vi "ConvertTextBasedCodeToLabVIEW_CreateInterfaceList.vi"(11 "Classes":T1[](array[typedef])) -> (3 "InterfaceItems":T13[](array[typedef]))   [LabVIEW 2020]
uses:
  ConvertTextBasedCodeToLabVIEW_MissingType.ctl
  ConvertTextBasedCodeToLabVIEW_MissingTypeIconType.ctl
  String/GDSString_ClassDescriptionType.ctl
  String/GDSString_AccessScopeModifierType.ctl
  String/GDSString_ModifierType.ctl
  String/GDSString_MethodDescriptionType.ctl
  CommonVIs/CommonVIs_AttributeType.ctl
  CommonVIs/CommonVIs_AttributeDataType.ctl
  CommonVIs/CommonVIs_PropertyType.ctl
  String/GDSString_ClassParentType.ctl
  String/GDSString_ClassType.ctl
  String/GDSString_ClassOwnerType.ctl
  CommonVIs/CommonVIs_EnumType.ctl
  CommonVIs/CommonVIs_StructType.ctl
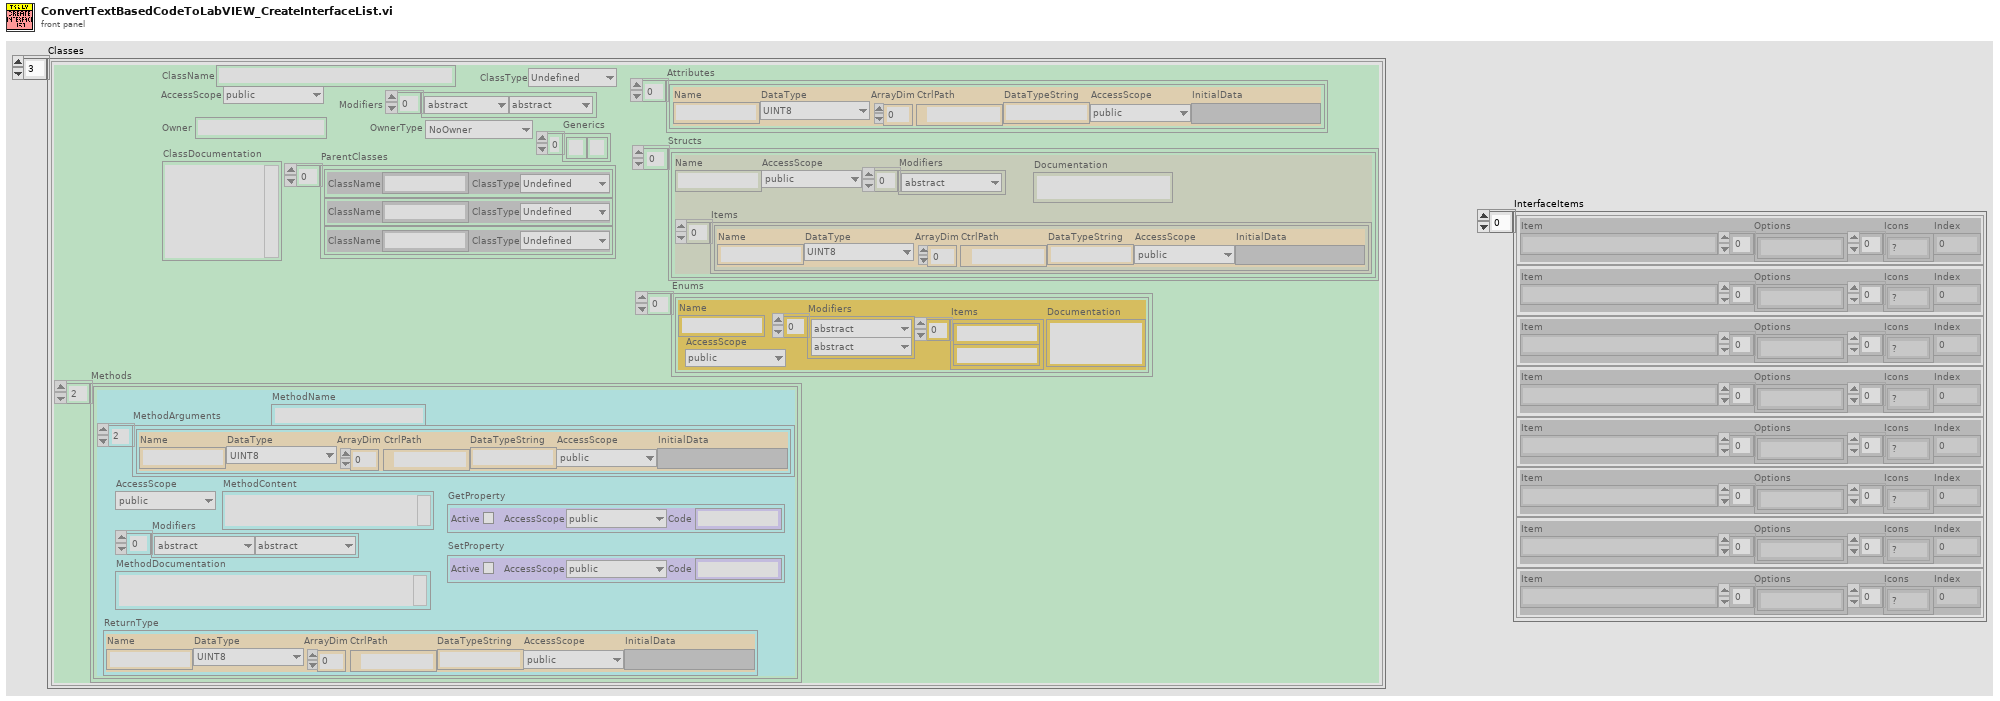
[diagram p1: front panel]
types:
  T1 = typedef "GDSString_ClassDescriptionType.ctl" = cluster{"ClassName":string, "AccessScope":T2, "Modifiers":T3[], "ClassDocumentation":string, "Methods":T4[], "ParentClasses":T8[], "ClassType":T9, "Owner":string, "OwnerType":T10, "Generics":string[], "Attributes":T5[], "Enums":T11[], "Structs":T12[]}
  T2 = typedef "GDSString_AccessScopeModifierType.ctl" = enum16{"public", "private", "protected", "internal"}
  T3 = typedef "GDSString_ModifierType.ctl" = enum16{"abstract", "static", "final", "synchronized", "strictfp", "async", "const", "event", "extern", "new", "native ", "override", "partial", "readonly", "sealed", "unsafe", "virtual", "volatile"}
  T4 = typedef "GDSString_MethodDescriptionType.ctl" = cluster{"ReturnType":T5, "MethodName":string, "AccessScope":T2, "Modifiers":T3[], "MethodDocumentation":string, "MethodContent":string, "MethodArguments":T5[], "GetProperty":T7, "SetProperty":T7}
  T5 = typedef "CommonVIs_AttributeType.ctl" = cluster{"Name":string, "DataType":T6, "ArrayDim":i32, "CtrlPath":path, "DataTypeString":string, "AccessScope":T2, "InitialData":variant}
  T6 = typedef "CommonVIs_AttributeDataType.ctl" = enum16{"UINT8", "INT8", "UINT16", "INT16", "UINT32", "INT32", "UINT64", "INT64", "SGL", "DBL", "EXT", "CSG", "CDB", "CXT", "TimeStamp", "STRING", "PATH", "BOOL", "ENUM", "RefNum", "VIRefNum", "LabVIEW Class", "Cluster", "Variant", "TypeDef", "Waveform", "LabVIEW Object", "Other", "void", "Set", "Map"}
  T7 = typedef "CommonVIs_PropertyType.ctl" = cluster{"Active":bool, "AccessScope":T2, "Code":string}
  T8 = typedef "GDSString_ClassParentType.ctl" = cluster{"ClassName":string, "ClassType":T9}
  T9 = typedef "GDSString_ClassType.ctl" = enum16{"Undefined", "Class", "Interface"}
  T10 = typedef "GDSString_ClassOwnerType.ctl" = enum16{"NoOwner", "Class", "Package/NameSpace"}
  T11 = typedef "CommonVIs_EnumType.ctl" = cluster{"Name":string, "AccessScope":T2, "Modifiers":T3[], "Items":string[], "Documentation":string}
  T12 = typedef "CommonVIs_StructType.ctl" = cluster{"Name":string, "AccessScope":T2, "Modifiers":T3[], "Items":T5[], "Documentation":string}
  T13 = typedef "ConvertTextBasedCodeToLabVIEW_MissingType.ctl" = cluster{"Item":string, "Options":string[], "Icons":T14[], "Index":i32}
  T14 = typedef "ConvertTextBasedCodeToLabVIEW_MissingTypeIconType.ctl" = enum16{"?", "Add", "Delete", "Implement", "Inherit"}
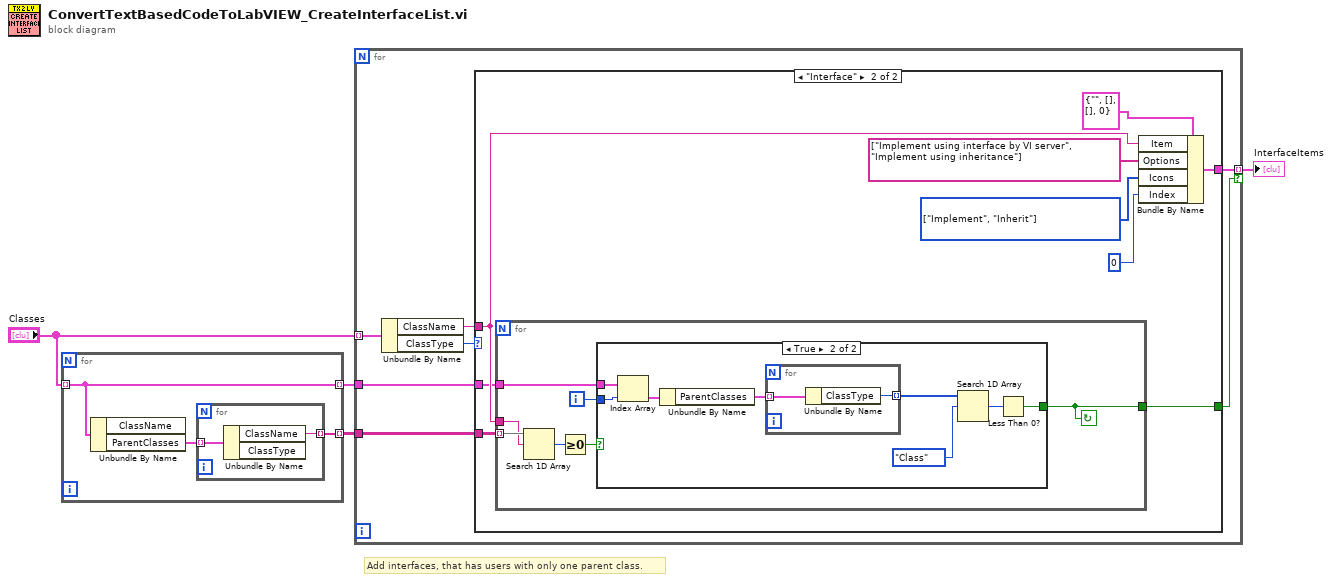
[diagram p0: block diagram]
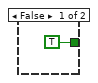
[diagram p3: hidden frame]
diagram:
  # "Add interfaces, that has users with only one parent class."
  n1 = for {
    tunnel: "Classes" -> [w5] mode=indexing
    tunnel: [w6] -> w3 mode=indexing
    tunnel: [w5] -> w2 mode=indexing
    n2 = Unbundle By Name(w5) -> ("ParentClasses"=w7:T8[])  [unwired: 1 out]
    n3 = for {
      tunnel: w7 -> [w9] mode=indexing
      tunnel: [w8] -> w6 mode=indexing
      n4 = Unbundle By Name(w9) -> ("ClassName"=w8:string)  [unwired: 1 out]
    }
  }
  n5 = for {
    tunnel: "Classes" -> [w16] mode=indexing
    tunnel: w3 -> [w13]
    tunnel: w2 -> [w12]
    tunnel: [w11] -> w1 mode=indexing if=w10
    n6 = Unbundle By Name(w16) -> ("ClassName"=w14:string, "ClassType"=w15:T9)
    n7 = case shown="\"Interface\"" w15 {
      tunnel: w14 -> [_ w20]
      tunnel: w13 -> [_ w21]
      tunnel: w12 -> [_ w19]
      tunnel: [_ w18] -> w11
      tunnel: [_ w17] -> w10
      frame Default {
      }
      frame "Interface" {
        w23 = T14[] [enum."Implement", enum."Inherit"] items=["?", "Add", "Delete", "Implement", "Inherit"] ("Icons")
        n8 = for {
          tunnel: w21 -> [w32] mode=indexing
          tunnel: w20 -> [w31]
          tunnel: w19 -> [w29]
          tunnel: [w26] -> w17
          i -> [w27]
          stop <- w26 continue-if-true
          n9 = Search 1D Array(1D array=w32, element=w31) -> (index of element=w28:i32)  [unwired: 1 in]
          n10 = Greater Or Equal To 0?(x=w28) -> (x >= 0?=w30:bool)
          n11 = case shown="True" w30 {
            tunnel: w29 -> [_ w41]
            tunnel: w27 -> [_ w40]
            tunnel: [TRUE w34] -> w26
            frame False {
            }
            frame True {
              n12 = Index Array(array=w41, index=w40) -> (element=w39:T1)
              n13 = Unbundle By Name(w39) -> ("ParentClasses"=w38:T8[])
              n14 = for {
                tunnel: w38 -> [w43] mode=indexing
                tunnel: [w42] -> w37 mode=indexing
                n15 = Unbundle By Name(w43) -> ("ClassType"=w42:T9)
              }
              n16 = Search 1D Array(1D array=w37, element=GDSString_ClassType."Class") -> (index of element=w35:i32)  [unwired: 1 in]
              n17 = Less Than 0?(x=w35) -> (x < 0?=w34:bool)
            }
          }
        }
        n18 = Bundle By Name(cluster=T13 {"Item"="", "Options"=[], "Icons"=[], "Index"=0} ("Cluster"), "Item"=w20, "Options"=string[] ["Implement using interface by VI server", "Implement using inheritance"], "Icons"=w23, "Index"=0 ("InitialIndex")) -> (w18:T13)
      }
    }
  }
  "InterfaceItems" <- w1
